vi "Run Sequence.vi"() -> ()   [LabVIEW 2019, in "Run Sequence.lvlib"]
uses:
  Run Sequence.lvlib
  support/States.ctl
  support/StateData.ctl
  <vilib>/Utility/miscctls.llb/LVRowAndColumnTypeDef.ctl
  <vilib>/Utility/sysdir.llb/System Directory Type.ctl
  <vilib>/Utility/file.llb/Read Delimited Spreadsheet (string).vi
  <vilib>/Utility/file.llb/Write Delimited Spreadsheet (string).vi
panel:
  in  "Refresh Button":bool
  in  "Open Sequences Folder":bool
  out "Sequence":string[][](table)
  in  "Select Sequence":i32(listbox)=-1
  in  "Run Sequence":bool
  # "Run Sequence"
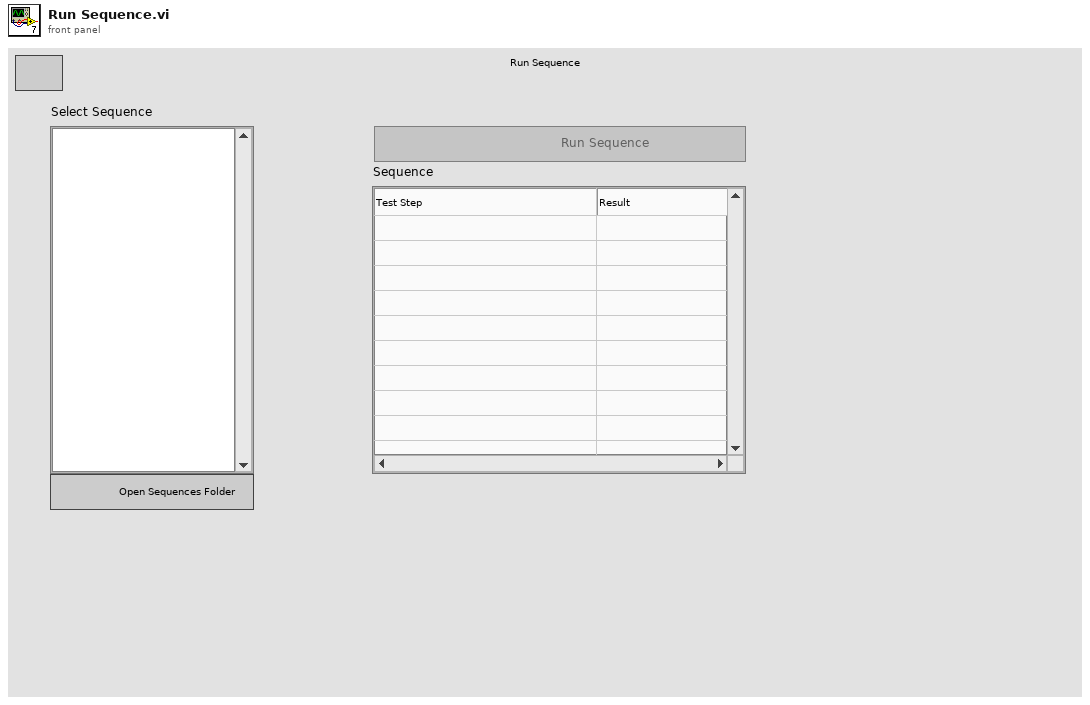
[diagram p1: front panel]
types:
  T1 = typedef "Run Sequence.lvlib/StateData.ctl" = cluster{"Sequence filepaths":path[], "Sequence table":string[][], "Sequence name":string, "Reports folder":path, "Sequences folder":path}
  T2 = typedef "Run Sequence.lvlib/States.ctl" = enum16{"Initialize", "Wait for Event", "Run Sequence", "Log Report File", "Shutdown"}
  T3 = typedef "LVRowAndColumnTypeDef.ctl" = cluster{"Row":i32, "Column":i32}
  T4 = enum8{"Enabled", "Disabled", "Disabled and Grayed Out"}
  T5 = typedef "System Directory Type.ctl" = i32
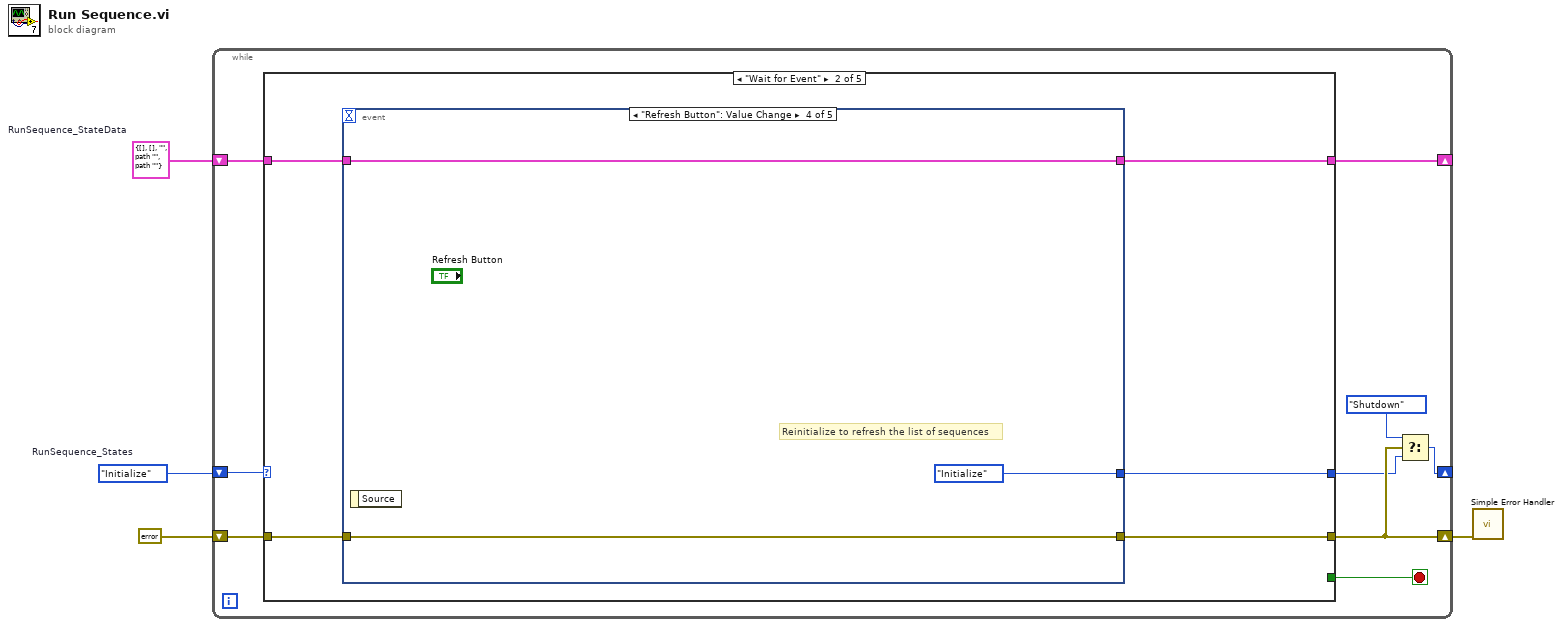
[diagram p0: block diagram]
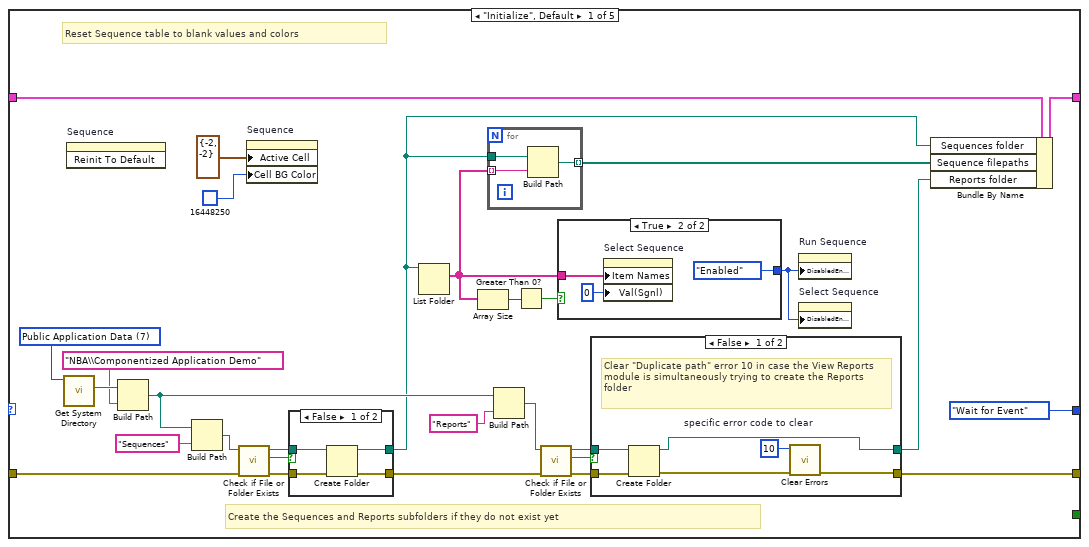
[diagram p2: hidden frame]
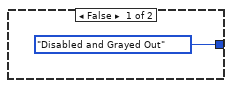
[diagram p3: hidden frame]
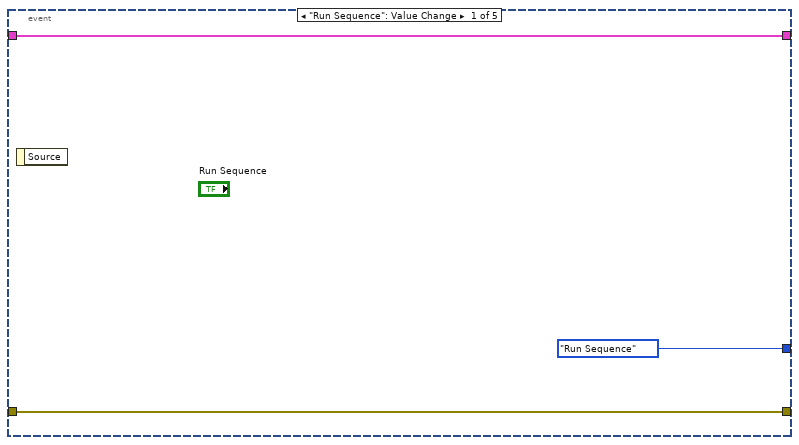
[diagram p6: hidden frame]
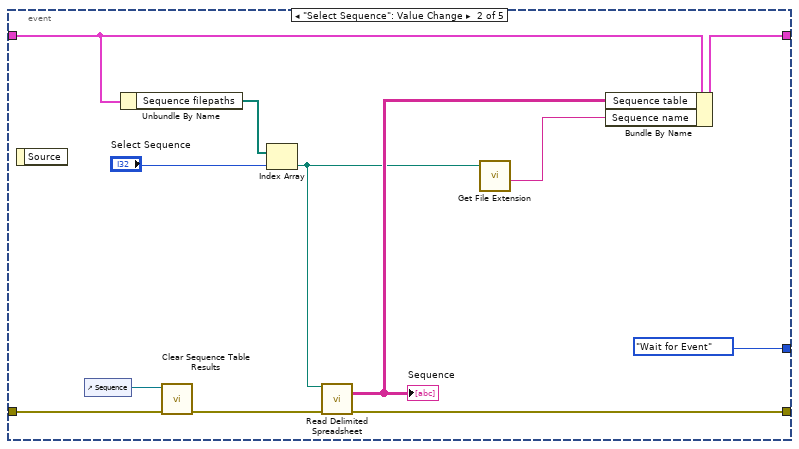
[diagram p7: hidden frame]
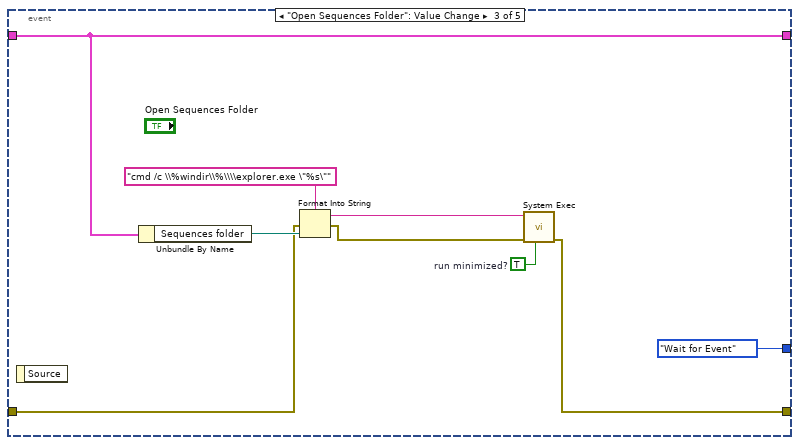
[diagram p8: hidden frame]
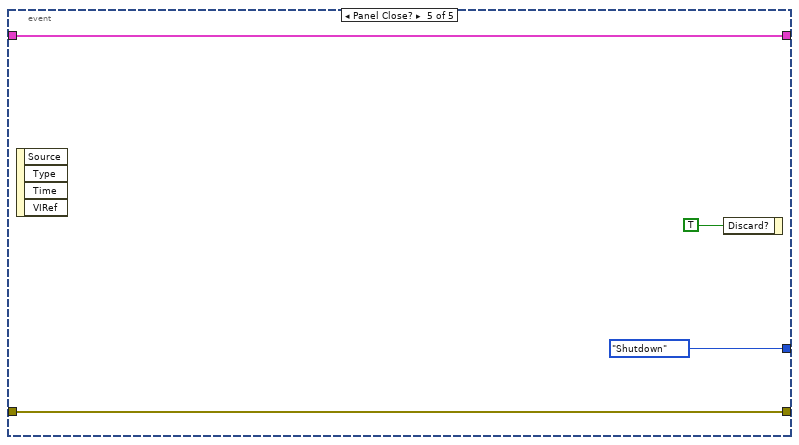
[diagram p9: hidden frame]
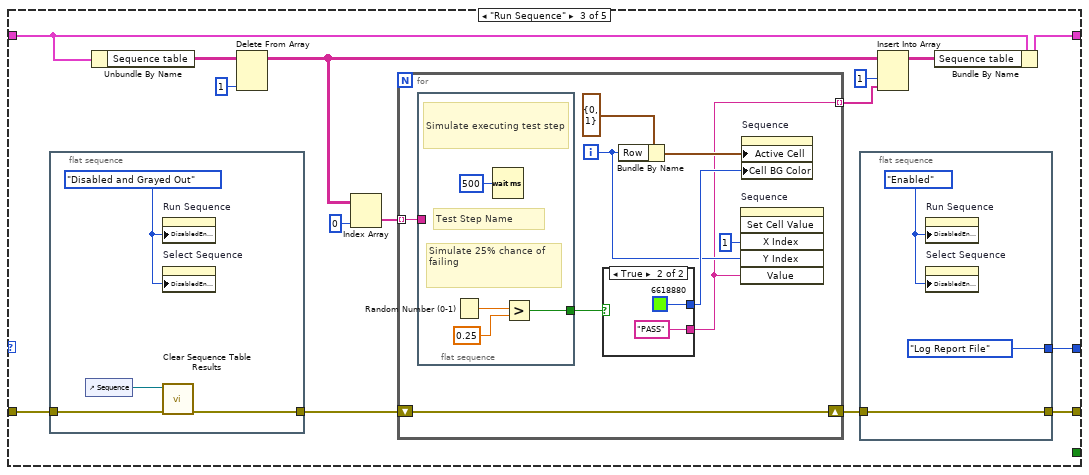
[diagram p10: hidden frame]
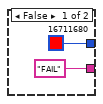
[diagram p11: hidden frame]
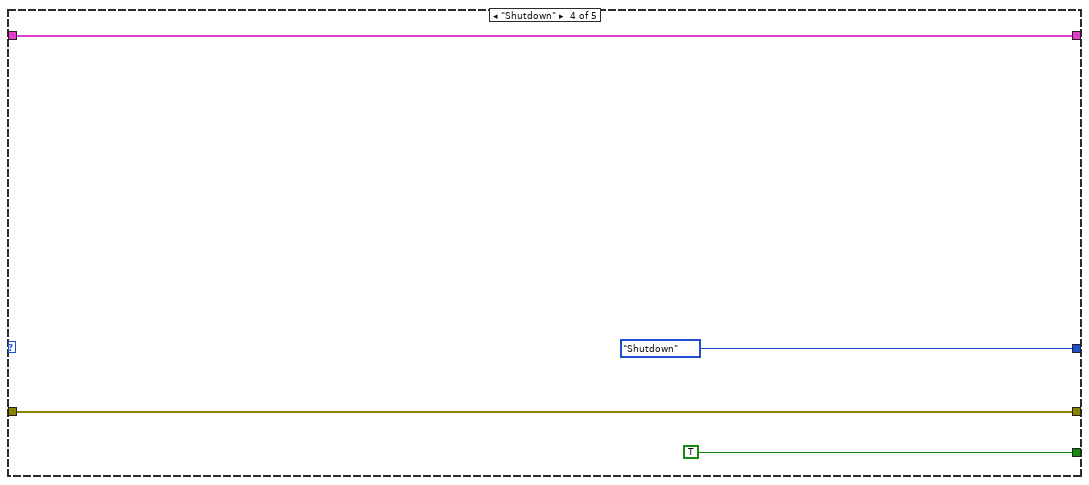
[diagram p12: hidden frame]
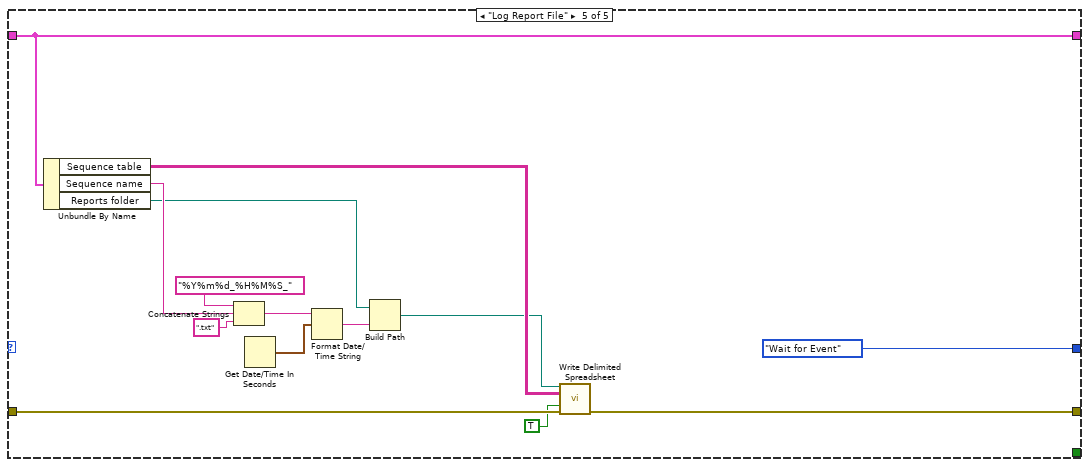
[diagram p13: hidden frame]
diagram:
  w3 = T1 {"Sequence filepaths"=[], "Sequence table"=[], "Sequence name"="", "Reports folder"=path "", "Sequences folder"=path ""}  # RunSequence_StateData
  w4 = States."Initialize"  # RunSequence_States
  n1 = while {
    shift-right: [w5] -> _
    shift-left: w4 -> [w13]
    shift-right: [w11] -> _
    shift-left: w3 -> [w12]
    shift-right: [w8] -> w1
    shift-left: errorcluster {"status"=FALSE, "code"=0, "source"=""} ("error in (no error)") -> [w9]
    stop <- w10 stop-if-true
    n2 = case shown="\"Wait for Event\"" w13 {
      tunnel: [States."Wait for Event" w68 w109 States."Shutdown" States."Wait for Event"] -> w7
      tunnel: w12 -> [w40 w67 w114 w142 w155]
      tunnel: [w39 w66 w105 w142 w155] -> w11
      tunnel: [_ _ _ TRUE _] -> w10
      tunnel: w9 -> [w25 w65 w111 w139 w156]
      tunnel: [w33 w64 w107 w139 w152] -> w8
      frame "Initialize", Default {
        w30 = T5 7 items=["User Home"=0, "User Desktop"=1, "User Documents"=2, "User Application Data"=3, "User Preferences"=4, "User Temporary"=5, "Public Documents"=6, "Public Application Data"=7, "Public Preferences"=8, "Public Cache"=13, "System Core Libraries"=9, "System Installed Libraries"=10, "Application Files"=11, "Boot Volume Root"=12] ("system directory type")
        # "Create the Sequences and Reports subfolders if they do not exist yet"
        # "Reset Sequence table to blank values and colors"
        n3 = call <vilib>:"Get System Directory.vi"("system directory type"=w30) -> ("system directory"=w22:path)  [unwired: 10 in]
        n4 = invoke on="Sequence" class="Tbl (strict)" method="Reinit To Default"() -> ()  [unwired: 3 in, 3 out]
        n5 = Build Path(base path=w22, name or relative path="NBA\\Componentized Application Demo") -> (appended path=w20:path)
        n6 = Build Path(base path=w20, name or relative path="Sequences") -> (appended path=w24:path)
        n7 = call <vilib>:"Check if File or Folder Exists.vi"("error in (no error)"=w25, "path"=w24) -> ("error out"=w26:errorcluster, "file or folder exists?"=w27:bool, "dup path"=w28:path)  [unwired: 7 in]
        n8 = property on="Sequence" class="Tbl (strict)"("Active Cell"=T3 {"Row"=-2, "Column"=-2} ("Active Cell:Active Cell"), "Cell BG Color"=u32 16448250) -> ()  [unwired: 2 in, 2 out]
        n9 = case shown="False" w27 {
          tunnel: w26 -> [w49 w52]
          tunnel: [w50 w52] -> w23
          tunnel: w28 -> [w48 w51]
          tunnel: [w47 w51] -> w14
          frame False {
            n10 = Create Folder(path (use dialog)=w48, error in=w49) -> (created path=w47:path, error out=w50:errorcluster)  [unwired: 1 in, 1 out]
          }
          frame True {
          }
        }
        n11 = List Folder(path=w14) -> (filenames=w19:string[])  [unwired: 3 in, 3 out]
        n12 = Array Size(array=w19) -> (size(s)=w18:i32)
        n13 = for {
          tunnel: w14 -> [w63]
          tunnel: w19 -> [w62] mode=indexing
          tunnel: [w61] -> w38 mode=indexing
          n14 = Build Path(base path=w63, name or relative path=w62) -> (appended path=w61:path)
        }
        n15 = Build Path(base path=w20, name or relative path="Reports") -> (appended path=w35:path)
        n16 = Greater Than 0?(x=w18) -> (x > 0?=w17:bool)
        n17 = call <vilib>:"Check if File or Folder Exists.vi"("error in (no error)"=w23, "path"=w35) -> ("error out"=w34:errorcluster, "file or folder exists?"=w32:bool, "dup path"=w31:path)  [unwired: 7 in]
        n18 = case shown="True" w17 {
          tunnel: w19 -> [_ w45]
          tunnel: [T4."Disabled and Grayed Out" ("Disabled") T4."Enabled" ("Disabled")] -> w16
          frame False {
          }
          frame True {
            n19 = property on="Select Sequence" class="LstBox (strict)"("Item Names"=w45, "Val(Sgnl)"=0 ("Select Sequence")) -> ()  [unwired: 2 in, 2 out]
          }
        }
        n20 = case shown="False" w32 {
          tunnel: w34 -> [w58 w60]
          tunnel: [w53 w60] -> w33
          tunnel: w31 -> [w57 w59]
          tunnel: [w56 w59] -> w15
          frame False {
            w55 = 10  # specific error code to clear
            # "Clear \"Duplicate path\" error 10 in case the View Reports module is simultaneously trying to create the Reports folder"
            n21 = Create Folder(path (use dialog)=w57, error in=w58) -> (created path=w56:path, error out=w54:errorcluster)  [unwired: 1 in, 1 out]
            n22 = call <vilib>:"Clear Errors.vi"("error in (no error)"=w54, "specific error code to clear (0: all)"=w55) -> ("error out"=w53:errorcluster)  [unwired: 4 in, 1 out]
          }
          frame True {
          }
        }
        n23 = property on="Run Sequence" class="Bool"("DisabledEnum"=w16) -> ()  [unwired: 2 in, 2 out]
        n24 = property on="Select Sequence" class="LstBox (strict)"("DisabledEnum"=w16) -> ()  [unwired: 2 in, 2 out]
        n25 = Bundle By Name(cluster=w40, "Sequences folder"=w14, "Sequence filepaths"=w38, "Reports folder"=w15) -> (w39:T1)
      }
      frame "Wait for Event" {
        n26 = event shown="[3] \"Refresh Button\": Value Change" {
          selector: _ -> [_ _ _ _ _]
          dyn-events: _ -> [_ _ _ _ _]
          timeout: _ -> [_ _ _ _ _]
          tunnel: [States."Run Sequence" States."Wait for Event" States."Wait for Event" States."Initialize" States."Shutdown"] -> w68
          tunnel: w67 -> [w70 w83 w87 w95 w97]
          tunnel: [w70 w78 w87 w95 w97] -> w66
          tunnel: w65 -> [w69 w75 w86 w94 w96]
          tunnel: [w69 w74 w85 w94 w96] -> w64
          event "Run Sequence": Value Change {
            n27 = event-data() -> ()  [unwired: 1 in, 1 out]
          }
          event "Select Sequence": Value Change {
            n28 = event-data() -> ()  [unwired: 1 in, 1 out]
            n29 = control-ref of="Sequence"() -> (w77:refnum<vi>)
            n30 = Unbundle By Name(w83) -> ("Sequence filepaths"=w82:path[])
            n31 = call "Clear Sequence Table Results.vi"("error in (no error)"=w75, "table reference in"=w77) -> ("error out"=w76:errorcluster)  [unwired: 8 in, 1 out]
            n32 = Index Array(array=w82, index="Select Sequence") -> (element=w73:path)
            n33 = call-poly <vilib>:"Read Delimited Spreadsheet.vi"("file path (dialog if empty)"=w73, "error in (no error)"=w76) -> ("all rows"=w79:string[][], "error out"=w74:errorcluster)  [unwired: 8 in, 4 out]
            "Sequence" <- w79
            n34 = call <vilib>:"Get File Extension.vi"("file"=w73) -> ("filename without extension"=w72:string)  [unwired: 6 in, 4 out]
            n35 = Bundle By Name(cluster=w83, "Sequence table"=w79, "Sequence name"=w72) -> (w78:T1)
          }
          event "Open Sequences Folder": Value Change {
            w90 = TRUE  # run minimized?
            n36 = event-data() -> ()  [unwired: 1 in, 1 out]
            n37 = Unbundle By Name(w87) -> ("Sequences folder"=w89:path)
            n38 = Format Into String(format string="cmd /c \\%windir\\%\\\\explorer.exe \"%s\"" ("name or relative path"), error in=w86, w89) -> (resulting string=w91:string, error out=w88:errorcluster)  [unwired: 1 in]
            n39 = call <vilib>:"System Exec.vi"("run minimized? (F)"=w90, "error in (no error)"=w88, "command line"=w91) -> ("error out"=w85:errorcluster)  [unwired: 5 in, 3 out]
          }
          event "Refresh Button": Value Change {
            # "Reinitialize to refresh the list of sequences"
            n40 = event-data() -> ()  [unwired: 1 in, 1 out]
          }
          event Panel Close? {
            n41 = event-data() -> ()  [unwired: 1 in, 4 out]
            n42 = event-data("Discard?"=TRUE) -> ()  [unwired: 1 in, 1 out]
          }
        }
      }
      frame "Run Sequence" {
        n43 = flat-sequence {
          tunnel: w111 -> [w119]
          tunnel: [w118] -> w110
          frame #0 {
            w121 = T4."Disabled and Grayed Out" ("Disabled")
            n44 = control-ref of="Sequence"() -> (w120:refnum<vi>)
            n45 = property on="Run Sequence" class="Bool"("DisabledEnum"=w121) -> ()  [unwired: 2 in, 2 out]
            n46 = property on="Select Sequence" class="LstBox (strict)"("DisabledEnum"=w121) -> ()  [unwired: 2 in, 2 out]
            n47 = call "Clear Sequence Table Results.vi"("error in (no error)"=w119, "table reference in"=w120) -> ("error out"=w118:errorcluster)  [unwired: 8 in, 1 out]
          }
        }
        n48 = Unbundle By Name(w114) -> ("Sequence table"=w102:string[][])
        n49 = Delete From Array(array=w102, index (col)=1 ("disabled index (col)")) -> (array with subset deleted=w101:string[][])  [unwired: 2 in, 1 out]
        n50 = Index Array(array=w101, index (col)=0 ("disabled index (col)")) -> (element=w112:string[])  [unwired: 1 in]
        n51 = for {
          tunnel: w112 -> [w125] mode=indexing
          shift-right: [w123] -> w108
          shift-left: w110 -> [w123]
          tunnel: [w122] -> w106 mode=indexing
          i -> [w126]
          n52 = flat-sequence {
            tunnel: w125 -> [_]
            tunnel: [w131] -> w124
            frame #0 {
              # "Test Step Name"
              # "Simulate 25% chance of failing"
              # "Simulate executing test step"
              n53 = Random Number (0-1)() -> (number: 0 to 1=w133:dbl)
              n54 = Wait (ms)(milliseconds to wait=u32 500) -> ()  [unwired: 1 out]
              n55 = Greater?(x=w133, y=0.25) -> (0:w131:bool)
            }
          }
          n56 = case shown="True" w124 {
            tunnel: [u32 16711680 u32 6618880] -> w130
            tunnel: ["FAIL" ("Value") "PASS" ("Value")] -> w122
            frame False {
            }
            frame True {
            }
          }
          n57 = Bundle By Name(cluster=T3 {"Row"=0, "Column"=1} ("Active Cell:Active Cell"), "Row"=w126) -> (w128:T3)
          n58 = invoke on="Sequence" class="Tbl (strict)" method="Set Cell Value"("X Index"=1 ("Y Index"), "Y Index"=w126, "Value"=w122) -> ()  [unwired: 3 in, 6 out]
          n59 = property on="Sequence" class="Tbl (strict)"("Active Cell"=w128, "Cell BG Color"=w130) -> ()  [unwired: 2 in, 2 out]
        }
        n60 = flat-sequence {
          tunnel: [States."Log Report File"] -> w109
          tunnel: w108 -> [w115]
          tunnel: [w115] -> w107
          frame #0 {
            w117 = T4."Enabled" ("Disabled")
            n61 = property on="Run Sequence" class="Bool"("DisabledEnum"=w117) -> ()  [unwired: 2 in, 2 out]
            n62 = property on="Select Sequence" class="LstBox (strict)"("DisabledEnum"=w117) -> ()  [unwired: 2 in, 2 out]
          }
        }
        n63 = Insert Into Array(array=w101, index (col)=1 ("disabled index (col)"), new element=w106) -> (w104:string[][])  [unwired: 1 in]
        n64 = Bundle By Name(cluster=w114, "Sequence table"=w104) -> (w105:T1)
      }
      frame "Shutdown" {
      }
      frame "Log Report File" {
        n65 = Unbundle By Name(w155) -> ("Sequence table"=w151:string[][], "Sequence name"=w146:string, "Reports folder"=w143:path)
        n66 = Concatenate Strings("%Y%m%d_%H%M%S_" ("time format string (%c)"), w146, ".txt" ("element")) -> (w144:string)
        n67 = Get Date/Time In Seconds() -> (seconds since 1Jan1904=w154:timestamp)
        n68 = Format Date/Time String(time format string (%c)=w144, seconds (now)=w154) -> (date/time string=w153:string)  [unwired: 1 in]
        n69 = Build Path(base path=w143, name or relative path=w153) -> (appended path=w150:path)
        n70 = call-poly <vilib>:"Write Delimited Spreadsheet.vi"("file path (dialog if empty)"=w150, "2D data"=w151, "append to file? (new file:F)"=TRUE, "error in (no error)"=w156) -> ("error out"=w152:errorcluster)  [unwired: 10 in, 1 out]
      }
    }
    n71 = Select(t=States."Shutdown", s=w8, f=w7) -> (s? t:f=w5:T2)
  }
  n72 = call <vilib>:"Simple Error Handler.vi"("error in (no error)"=w1) -> ()  [unwired: 4 in, 5 out]
